vi "DSS-Tests-summary_r140.vi"(11 "R140 data":T1) -> (3 "summary":dbl[](array[numeric]))   [LabVIEW 2020, in "DSS-Tests.lvlib"]
doc: "Summarises an R140 data cluster as one 1D DBL array: for each of its seven arrays in cluster order, the length, the first and the last element."
uses:
  DSS-Tests.lvlib
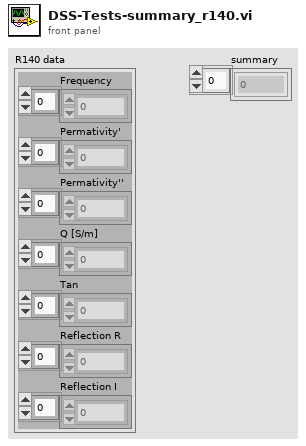
[diagram p1: front panel]
types:
  T1 = cluster{"Frequency":dbl[], "Permativity'":dbl[], "Permativity''":dbl[], "Q [S/m]":dbl[], "Tan":dbl[], "Reflection R":dbl[], "Reflection I":dbl[]}
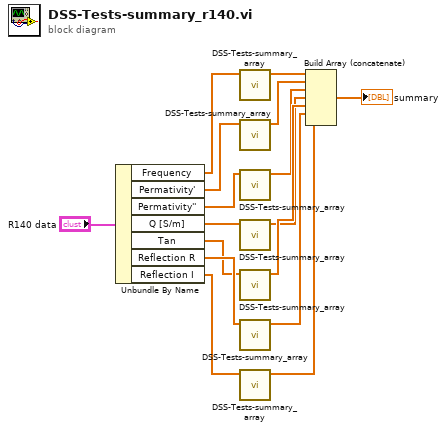
[diagram p0: block diagram]
diagram:
  n1 = Unbundle By Name("R140 data") -> ("Frequency"=w2:dbl[], "Permativity'"=w3:dbl[], "Permativity''"=w4:dbl[], "Q [S/m]"=w5:dbl[], "Tan"=w6:dbl[], "Reflection R"=w7:dbl[], "Reflection I"=w8:dbl[])
  n2 = call "DSS-Tests-summary_array.vi"("values"=w2) -> ("summary"=w9:dbl[])  [unwired: 10 in]
  n3 = call "DSS-Tests-summary_array.vi"("values"=w3) -> ("summary"=w10:dbl[])  [unwired: 10 in]
  n4 = call "DSS-Tests-summary_array.vi"("values"=w4) -> ("summary"=w11:dbl[])  [unwired: 10 in]
  n5 = call "DSS-Tests-summary_array.vi"("values"=w5) -> ("summary"=w12:dbl[])  [unwired: 10 in]
  n6 = call "DSS-Tests-summary_array.vi"("values"=w6) -> ("summary"=w13:dbl[])  [unwired: 10 in]
  n7 = call "DSS-Tests-summary_array.vi"("values"=w7) -> ("summary"=w14:dbl[])  [unwired: 10 in]
  n8 = call "DSS-Tests-summary_array.vi"("values"=w8) -> ("summary"=w15:dbl[])  [unwired: 10 in]
  n9 = Build Array (concatenate)(w9, w10, w11, w12, w13, w14, w15) -> (→"summary":dbl[])
